vi "Code Benchmark Template.vi"() -> ()   [LabVIEW 2017]
doc: "Use this template to build a VI to use as a subVI. This VI serves as a counter that counts the times that certain codes run in inner for loop and outer for loop."
panel:
  out "outside":i32
  out "inside":i32
  out "unit (ms)":dbl[](graph)
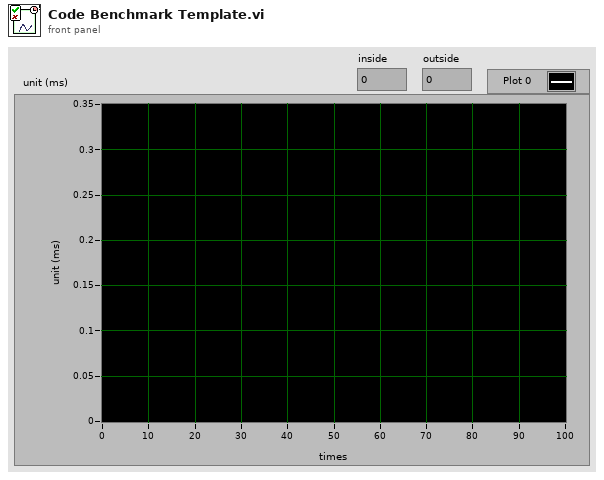
[diagram p1: front panel]
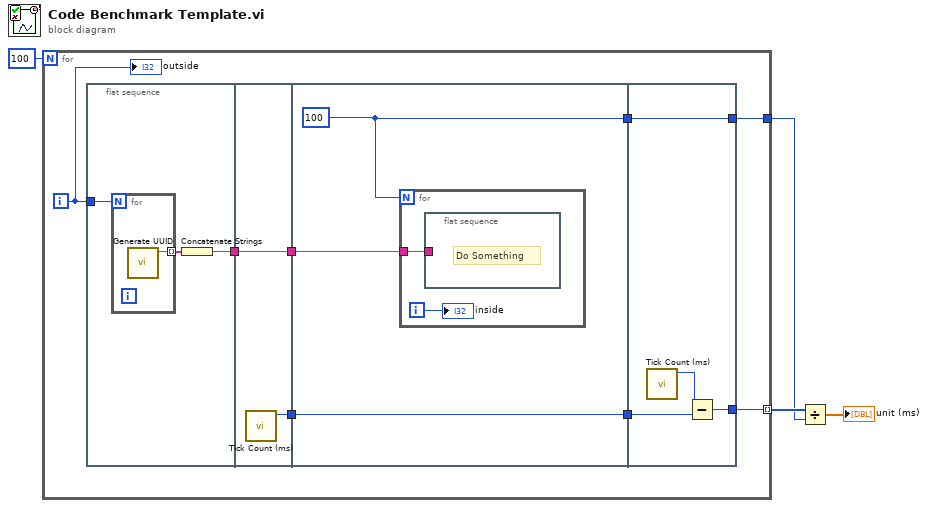
[diagram p0: block diagram]
diagram:
  n1 = for {
    N: 100 -> [_]
    tunnel: [w10] -> w2 mode=indexing
    tunnel: [w9] -> w1
    i -> [w5]
    n2 = flat-sequence {
      tunnel: w5 -> [w15]
      tunnel: [w13] -> w6
      tunnel: [w18] -> w12
      tunnel: [w17] -> w7
      tunnel: w6 -> [w17]
      tunnel: w12 -> [w21]
      tunnel: [w21] -> w11
      tunnel: [w20] -> w8
      tunnel: w7 -> [w19]
      tunnel: w11 -> [w26]
      tunnel: [w25] -> w10
      tunnel: [w24] -> w9
      tunnel: w8 -> [w24]
      frame #0 {
        n3 = for {
          N: w15 -> [_]
          tunnel: [w16] -> w14 mode=indexing
          n4 = call "Generate UUID.vi"() -> ("UUID"=w16:string)  [unwired: 11 in]
        }
        n5 = Concatenate Strings(w14) -> (w13:string)
      }
      frame #1 {
        n6 = call "Tick Count (ms).vi"() -> ("millisecond timer value"=w18:u32)  [unwired: 10 in, 1 out]
      }
      frame #2 {
        w20 = 100
        n7 = for {
          N: w20 -> [_]
          tunnel: w19 -> [w22]
          i -> [w23]
          n8 = flat-sequence {
            tunnel: w22 -> [_]
            frame #0 {
              # "Do Something"
            }
          }
          "inside" <- w23
        }
      }
      frame #3 {
        n9 = call "Tick Count (ms).vi"() -> ("millisecond timer value"=w27:u32)  [unwired: 10 in, 1 out]
        n10 = Subtract(x=w27, y=w26) -> (x-y=w25:u32)
      }
    }
    "outside" <- w5
  }
  n11 = Divide(x=w2, y=w1) -> (x/y=→"unit (ms)":dbl[])
